vi "CIF_CIPC_Tag Update Test Cases.vi"() -> (0 "error out":errorcluster, 2 "status":string, 3 "pass":bool)   [LabVIEW 2021]
uses:
  <vilib>/CIF Foundation/CIF Channels Core/ChannelCommon/typedef/Direction.ctl
  Double/CIF_CIPC_Chn_Double.lvclass
  C:/Program Files/National Instruments/LabVIEW 2021/vi.lib/CIF Foundation/CIF Channels Core/CIFChannels/CIFChannels.lvclass
  <vilib>/CIF Foundation/CIF Channels Core/ChannelCommon/typedef/New FIFO Instance Response.ctl
  U64/CIF_CIPC_Chn_U64.lvclass
  I64/CIF_CIPC_Chn_I64.lvclass
  a89bac37-e40b-4e23-8b15-caa5b580b70d.vi
  5767d73f-78c6-4091-81b3-8b4b134aad93.vi
  e629907d-3875-4979-a690-95404f934dc5.vi
  a89bac37-e40b-4e23-8b15-caa5b580b70d.vi/49b3dd2d-4579-4089-b72e-3f0875c862f2.vi
  <vilib>/CIF Foundation/CIF CIPC/SubVIs/Check Error.vi
  <vilib>/CIF Foundation/CIF CIPC/SubVIs/Add CIPC Error.vi
  <vilib>/CIF Foundation/CIF CIPC/SubVIs/Get dll Path.vi
  <vilib>/CIF Foundation/CIF CIPC/SubVIs/Notify Of New Write.vi
  <vilib>/CIF Foundation/CIF CIPC/SubVIs/Get Element Write Position.vi
  <vilib>/CIF Foundation/CIF CIPC/SubVIs/Wait For N Elements Available.vi
  <vilib>/CIF Foundation/CIF CIPC/SubVIs/Get Element Read Position.vi
  <vilib>/CIF Foundation/CIF CIPC/SubVIs/Set Element Read Position.vi
  <vilib>/CIF Foundation/CIF CIPC/SubVIs/Get Element Description Variant.vi
  <vilib>/Utility/error.llb/Trim Whitespace.vi
  <vilib>/CIF Foundation/CIF CIPC/SubVIs/Check Error Core.vi
  <vilib>/CIF Foundation/CIF CIPC/SubVIs/Add CIPC Error Core.vi
  <vilib>/CIF Foundation/CIF CIPC/SubVIs/Get Element Info Variant.vi
  <vilib>/CIF Foundation/CIF Channels Core/ChannelCommon/ChannelCommon.lvlib
  <vilib>/CIF Foundation/CIF Channels Core/CIFChannels/CIFChannels.lvclass
  <vilib>/CIF Foundation/CIF CIPC/CIF_NI_CIPC.lvlib
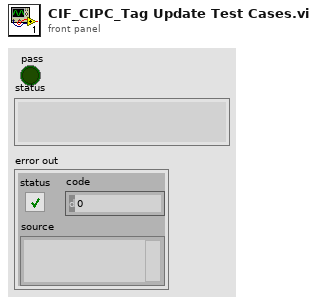
[diagram p1: front panel]
types:
  T1 = typedef "ChannelCommon.lvlib/Direction.ctl" = enum8{"Publisher", "Subscriber"}
  T2 = typedef "ChannelCommon.lvlib/New FIFO Instance Response.ctl" = cluster{"Publisher":string, "Custom Data":u8[]}
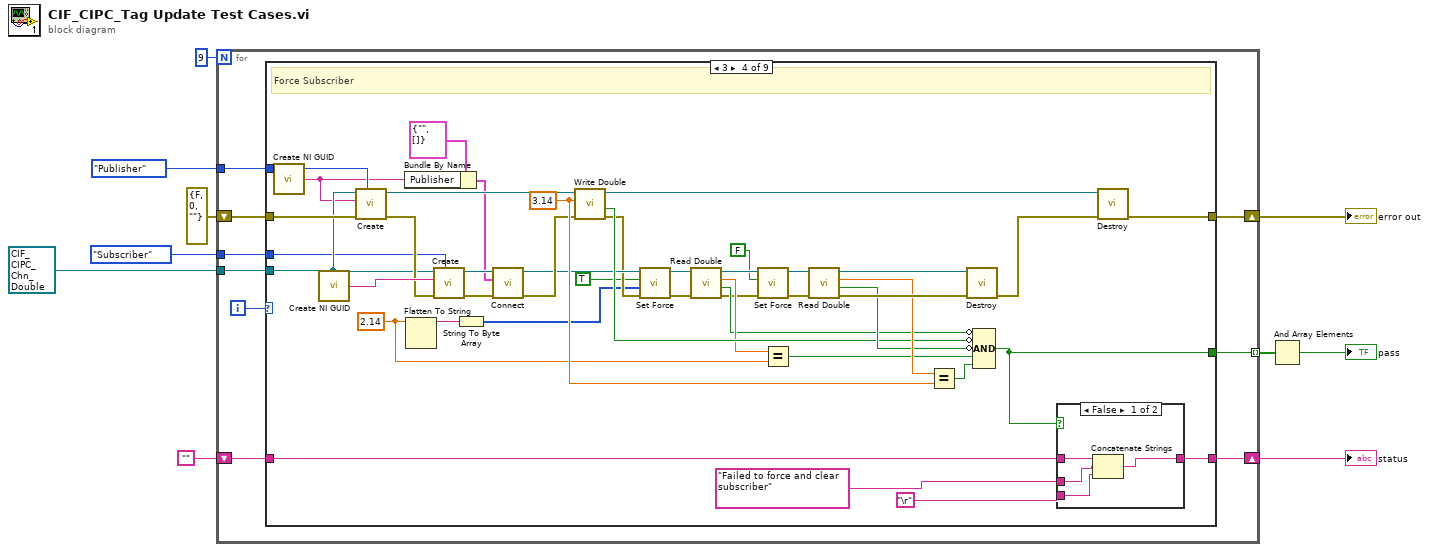
[diagram p0: block diagram]
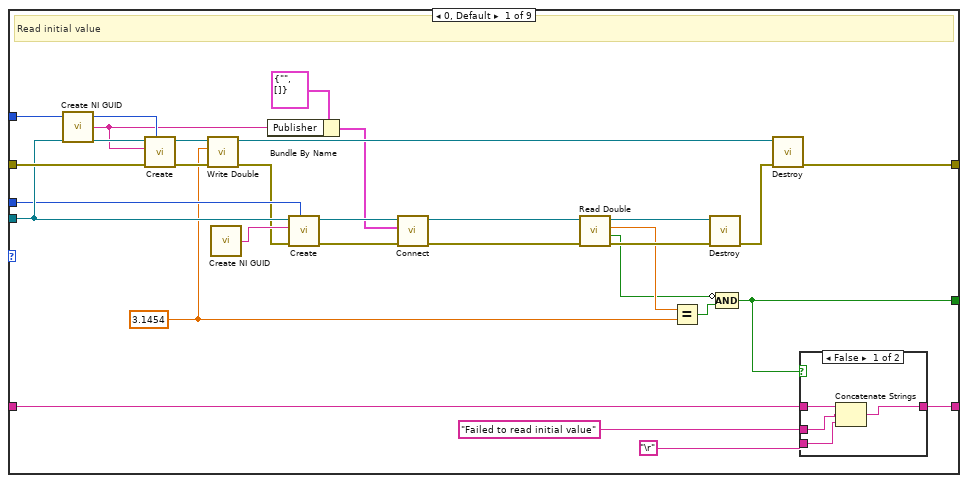
[diagram p2: hidden frame]
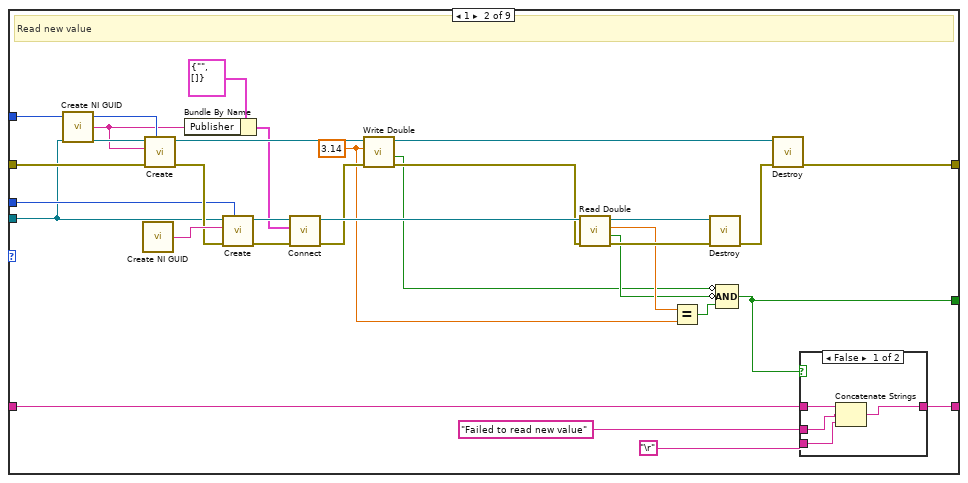
[diagram p4: hidden frame]
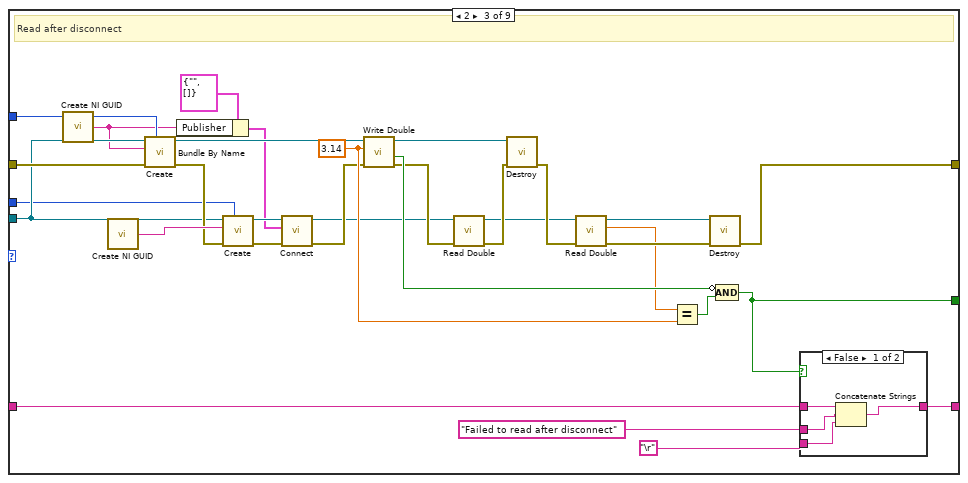
[diagram p6: hidden frame]
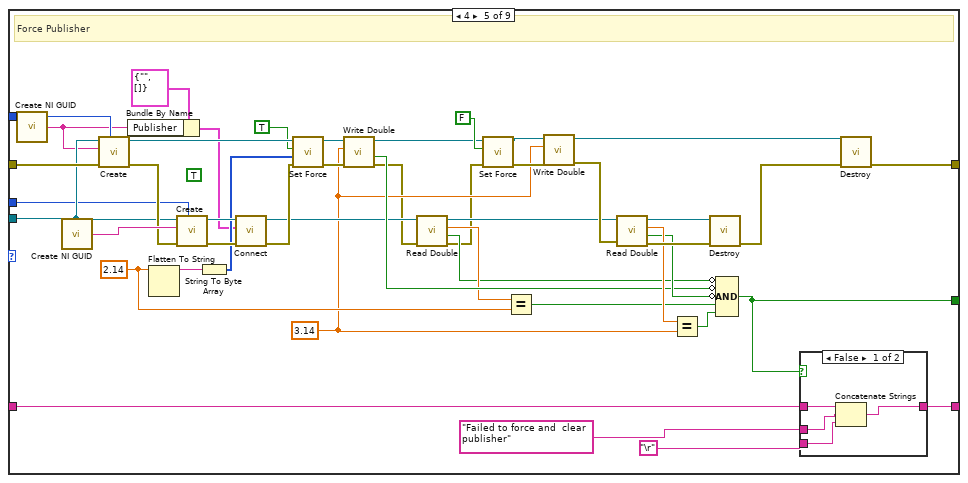
[diagram p9: hidden frame]
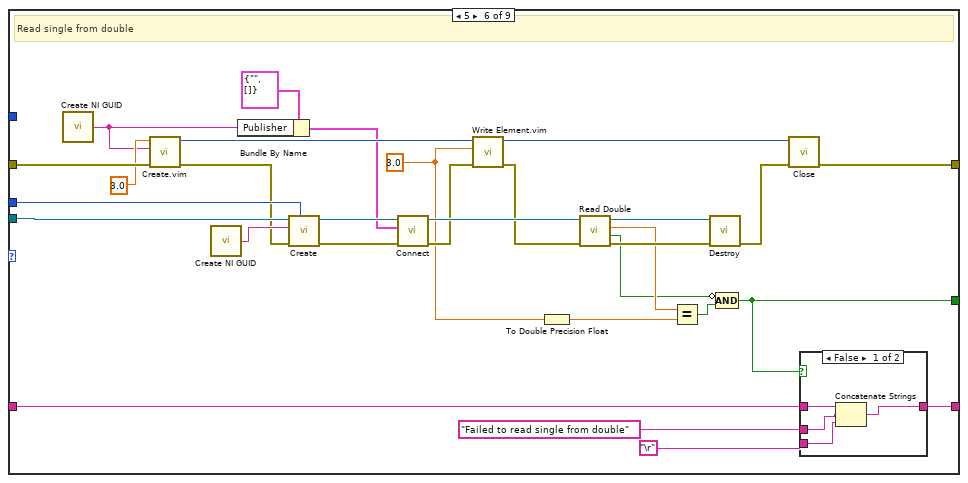
[diagram p11: hidden frame]
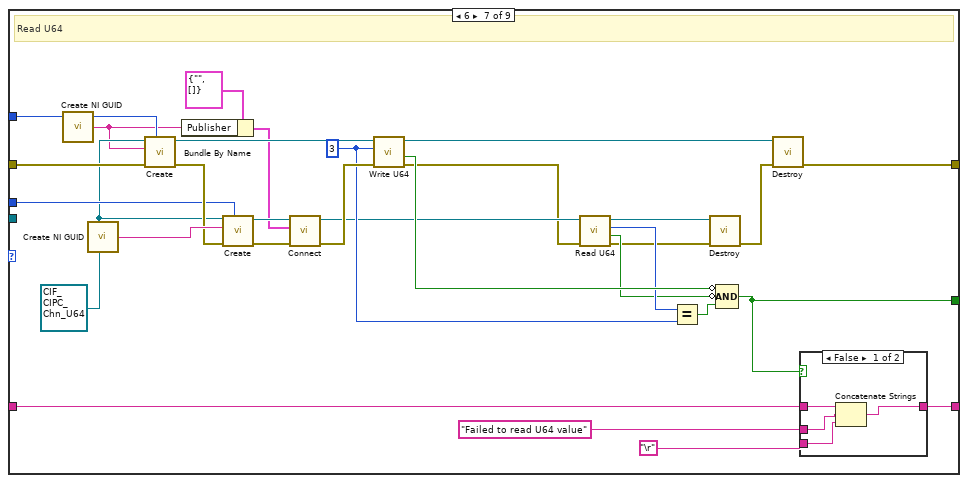
[diagram p13: hidden frame]
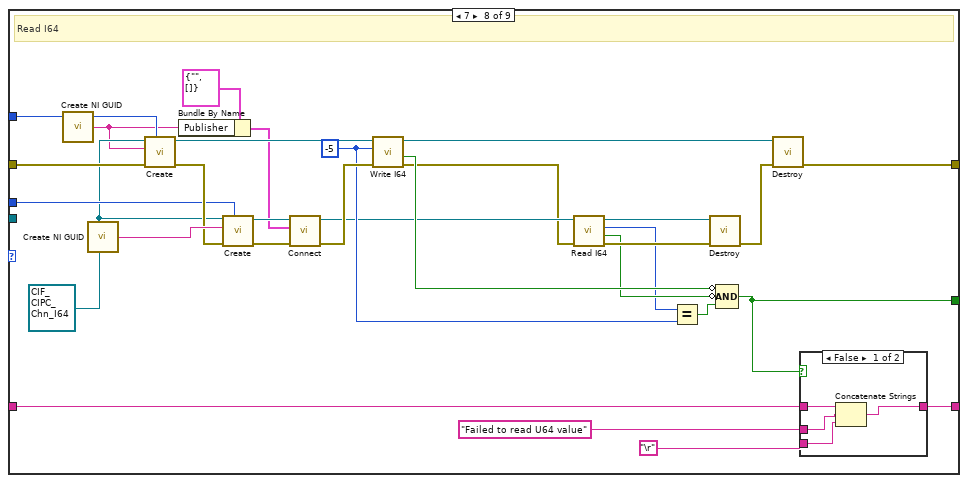
[diagram p15: hidden frame]
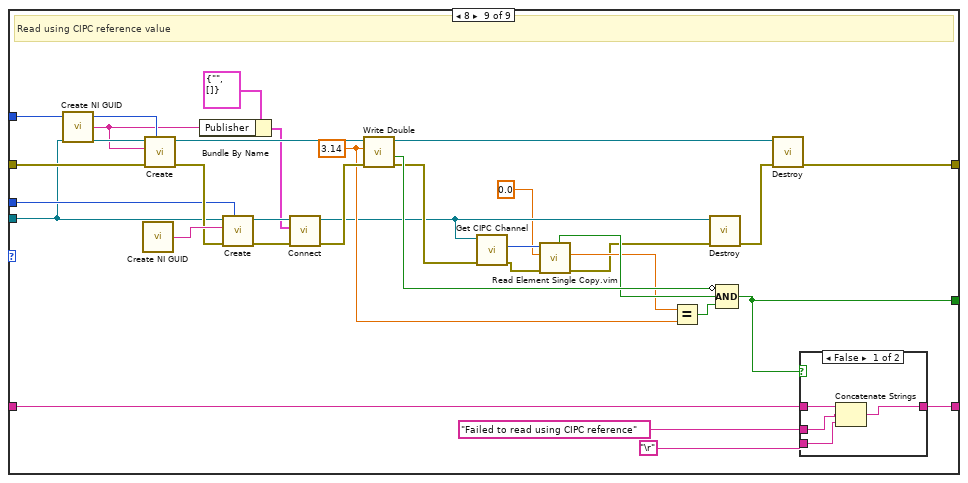
[diagram p17: hidden frame]
diagram:
  n1 = for {
    N: 9 -> [_]
    tunnel: [w19] -> w10 mode=indexing
    shift-right: [w17] -> w5
    shift-left: errorcluster {"status"=FALSE, "code"=0, "source"=""} ("error out") -> [w18]
    shift-right: [w14] -> w6
    shift-left: "" -> [w15]
    tunnel: refnum<class "CIF_CIPC_Chn_Double.lvclass"> refnum ("CIF_CIPC_Chn_Double.lvclass") -> [w13]
    tunnel: Direction."Publisher" ("Direction") -> [w12]
    tunnel: Direction."Subscriber" ("Direction") -> [w11]
    i -> [w16]
    n2 = case shown="3" w16 {
      tunnel: [w32 w67 w111 w158 w209 w242 w277 w312 w349] -> w19
      tunnel: w18 -> [w44 w79 w115 w164 w215 w234 w285 w320 w357]
      tunnel: [w35 w70 w104 w128 w193 w237 w279 w314 w351] -> w17
      tunnel: w15 -> [w48 w83 w119 w168 w219 w254 w289 w324 w361]
      tunnel: [w47 w82 w118 w167 w218 w253 w288 w323 w360] -> w14
      tunnel: w13 -> [w29 w57 w99 w149 w204 w240 _ _ w341]
      tunnel: w12 -> [w30 w59 w98 w148 w203 _ w276 w311 w343]
      tunnel: w11 -> [w28 w58 w97 w147 w202 w239 w275 w310 w342]
      frame 0, Default {
        w23 = 3.1454
        # "Read initial value"
        n3 = call <vilib>:"Create NI GUID.vi"() -> ("NI GUID"=w21:string)
        n4 = call-dynamic "Create.vi"("Direction"=w30, "error in (no error)"=w44, "Name"=w21, "CIFTag in"=w29) -> ("error out"=w26:errorcluster, "CIFTag out"=w27:refnum<class "CIF_CIPC_Chn_Double.lvclass">)  [unwired: 6 in]
        n5 = call-dynamic "Write Double.vi"("error in (no error)"=w26, "Data"=w23, "CIFTag in"=w27) -> ("error out"=w24:errorcluster, "CIFTag out"=w25:refnum<class "CIF_CIPC_Chn_Double.lvclass">)  [unwired: 6 in, 1 out]
        n6 = call <vilib>:"Create NI GUID.vi"() -> ("NI GUID"=w43:string)
        n7 = Bundle By Name(cluster=T2 {"Publisher"="", "Custom Data"=[]} ("Connection"), "Publisher"=w21) -> (w20:T2)
        n8 = call-dynamic "Create.vi"("Direction"=w28, "error in (no error)"=w24, "Name"=w43, "CIFTag in"=w29) -> ("error out"=w41:errorcluster, "CIFTag out"=w42:refnum<class "CIF_CIPC_Chn_Double.lvclass">)  [unwired: 6 in]
        n9 = call-dynamic "Connect.vi"("error in (no error)"=w41, "Connection"=w20, "CIFTag in"=w42) -> ("error out"=w39:errorcluster, "CIFTag out"=w40:refnum<class "CIF_CIPC_Chn_Double.lvclass">)  [unwired: 7 in]
        n10 = call-dynamic "Read Double.vi"("error in (no error)"=w39, "CIFTag in"=w40) -> ("error out"=w37:errorcluster, "timed out?"=w31:bool, "Data"=w34:dbl, "CIFTag out"=w38:refnum<class "CIF_CIPC_Chn_Double.lvclass">)  [unwired: 6 in]
        n11 = Equal?(x=w34, y=w23) -> (x = y?=w33:bool)
        n12 = call-dynamic "Destroy.vi"("error in (no error)"=w37, "CIFTag in"=w38) -> ("error out"=w36:errorcluster)  [unwired: 8 in, 1 out]
        n13 = Compound Arithmetic op=AND(invert w31, w33) -> (w32:bool)
        n14 = call-dynamic "Destroy.vi"("error in (no error)"=w36, "CIFTag in"=w25) -> ("error out"=w35:errorcluster)  [unwired: 8 in, 1 out]
        n15 = case shown="False" w32 {
          tunnel: w48 -> [w52 w53]
          tunnel: [w49 w53] -> w47
          tunnel: "Failed to read initial value" -> [w51 _]
          tunnel: "\r" -> [w50 _]
          frame False {
            n16 = Concatenate Strings(w52, w51, w50) -> (w49:string)
          }
          frame True {
          }
        }
      }
      frame 1 {
        w60 = 3.14 ("Data")
        # "Read new value"
        n17 = call <vilib>:"Create NI GUID.vi"() -> ("NI GUID"=w55:string)
        n18 = call <vilib>:"Create NI GUID.vi"() -> ("NI GUID"=w78:string)
        n19 = call-dynamic "Create.vi"("Direction"=w59, "error in (no error)"=w79, "Name"=w55, "CIFTag in"=w57) -> ("error out"=w77:errorcluster, "CIFTag out"=w65:refnum<class "CIF_CIPC_Chn_Double.lvclass">)  [unwired: 6 in]
        n20 = Bundle By Name(cluster=T2 {"Publisher"="", "Custom Data"=[]} ("Connection"), "Publisher"=w55) -> (w54:T2)
        n21 = call-dynamic "Create.vi"("Direction"=w58, "error in (no error)"=w77, "Name"=w78, "CIFTag in"=w57) -> ("error out"=w75:errorcluster, "CIFTag out"=w76:refnum<class "CIF_CIPC_Chn_Double.lvclass">)  [unwired: 6 in]
        n22 = call-dynamic "Connect.vi"("error in (no error)"=w75, "Connection"=w54, "CIFTag in"=w76) -> ("error out"=w64:errorcluster, "CIFTag out"=w74:refnum<class "CIF_CIPC_Chn_Double.lvclass">)  [unwired: 7 in]
        n23 = call-dynamic "Write Double.vi"("error in (no error)"=w64, "Data"=w60, "CIFTag in"=w65) -> ("error out"=w63:errorcluster, "timed out?"=w61:bool, "CIFTag out"=w62:refnum<class "CIF_CIPC_Chn_Double.lvclass">)  [unwired: 6 in]
        n24 = call-dynamic "Read Double.vi"("error in (no error)"=w63, "CIFTag in"=w74) -> ("error out"=w72:errorcluster, "timed out?"=w66:bool, "Data"=w69:dbl, "CIFTag out"=w73:refnum<class "CIF_CIPC_Chn_Double.lvclass">)  [unwired: 6 in]
        n25 = Equal?(x=w69, y=w60) -> (x = y?=w68:bool)
        n26 = call-dynamic "Destroy.vi"("error in (no error)"=w72, "CIFTag in"=w73) -> ("error out"=w71:errorcluster)  [unwired: 8 in, 1 out]
        n27 = Compound Arithmetic op=AND(invert w61, invert w66, w68) -> (w67:bool)
        n28 = call-dynamic "Destroy.vi"("error in (no error)"=w71, "CIFTag in"=w62) -> ("error out"=w70:errorcluster)  [unwired: 8 in, 1 out]
        n29 = case shown="False" w67 {
          tunnel: w83 -> [w87 w88]
          tunnel: [w84 w88] -> w82
          tunnel: "Failed to read new value" -> [w86 _]
          tunnel: "\r" -> [w85 _]
          frame False {
            n30 = Concatenate Strings(w87, w86, w85) -> (w84:string)
          }
          frame True {
          }
        }
      }
      frame 2 {
        w105 = 3.14 ("Data")
        # "Read after disconnect"
        n31 = call <vilib>:"Create NI GUID.vi"() -> ("NI GUID"=w90:string)
        n32 = call <vilib>:"Create NI GUID.vi"() -> ("NI GUID"=w114:string)
        n33 = call-dynamic "Create.vi"("Direction"=w98, "error in (no error)"=w115, "Name"=w90, "CIFTag in"=w99) -> ("error out"=w113:errorcluster, "CIFTag out"=w110:refnum<class "CIF_CIPC_Chn_Double.lvclass">)  [unwired: 6 in]
        n34 = Bundle By Name(cluster=T2 {"Publisher"="", "Custom Data"=[]} ("Connection"), "Publisher"=w90) -> (w89:T2)
        n35 = call-dynamic "Create.vi"("Direction"=w97, "error in (no error)"=w113, "Name"=w114, "CIFTag in"=w99) -> ("error out"=w102:errorcluster, "CIFTag out"=w103:refnum<class "CIF_CIPC_Chn_Double.lvclass">)  [unwired: 6 in]
        n36 = call-dynamic "Connect.vi"("error in (no error)"=w102, "Connection"=w89, "CIFTag in"=w103) -> ("error out"=w101:errorcluster, "CIFTag out"=w100:refnum<class "CIF_CIPC_Chn_Double.lvclass">)  [unwired: 7 in]
        n37 = call-dynamic "Write Double.vi"("error in (no error)"=w101, "Data"=w105, "CIFTag in"=w110) -> ("error out"=w108:errorcluster, "timed out?"=w109:bool, "CIFTag out"=w107:refnum<class "CIF_CIPC_Chn_Double.lvclass">)  [unwired: 6 in]
        n38 = call-dynamic "Read Double.vi"("error in (no error)"=w108, "CIFTag in"=w100) -> ("error out"=w106:errorcluster, "CIFTag out"=w95:refnum<class "CIF_CIPC_Chn_Double.lvclass">)  [unwired: 6 in, 2 out]
        n39 = call-dynamic "Destroy.vi"("error in (no error)"=w106, "CIFTag in"=w107) -> ("error out"=w96:errorcluster)  [unwired: 8 in, 1 out]
        n40 = call-dynamic "Read Double.vi"("error in (no error)"=w96, "CIFTag in"=w95) -> ("error out"=w94:errorcluster, "Data"=w93:dbl, "CIFTag out"=w92:refnum<class "CIF_CIPC_Chn_Double.lvclass">)  [unwired: 6 in, 1 out]
        n41 = Equal?(x=w93, y=w105) -> (x = y?=w112:bool)
        n42 = call-dynamic "Destroy.vi"("error in (no error)"=w94, "CIFTag in"=w92) -> ("error out"=w104:errorcluster)  [unwired: 8 in, 1 out]
        n43 = Compound Arithmetic op=AND(invert w109, w112) -> (w111:bool)
        n44 = case shown="False" w111 {
          tunnel: w119 -> [w123 w124]
          tunnel: [w120 w124] -> w118
          tunnel: "Failed to read after disconnect" -> [w122 _]
          tunnel: "\r" -> [w121 _]
          frame False {
            n45 = Concatenate Strings(w123, w122, w121) -> (w120:string)
          }
          frame True {
          }
        }
      }
      frame 3 {
        w138 = 2.14 ("Data")
        w153 = 3.14 ("Data")
        # "Force Subscriber"
        n46 = call <vilib>:"Create NI GUID.vi"() -> ("NI GUID"=w126:string)
        n47 = call <vilib>:"Create NI GUID.vi"() -> ("NI GUID"=w163:string)
        n48 = call-dynamic "Create.vi"("Direction"=w148, "error in (no error)"=w164, "Name"=w126, "CIFTag in"=w149) -> ("error out"=w162:errorcluster, "CIFTag out"=w156:refnum<class "CIF_CIPC_Chn_Double.lvclass">)  [unwired: 6 in]
        n49 = Bundle By Name(cluster=T2 {"Publisher"="", "Custom Data"=[]} ("Connection"), "Publisher"=w126) -> (w125:T2)
        n50 = Flatten To String(anything=w138) -> (data string=w144:string)  [unwired: 3 in, 2 out]
        n51 = call-dynamic "Create.vi"("Direction"=w147, "error in (no error)"=w162, "Name"=w163, "CIFTag in"=w149) -> ("error out"=w151:errorcluster, "CIFTag out"=w152:refnum<class "CIF_CIPC_Chn_Double.lvclass">)  [unwired: 6 in]
        n52 = String To Byte Array(string=w144) -> (unsigned byte array=w143:u8[])
        n53 = call-dynamic "Connect.vi"("error in (no error)"=w151, "Connection"=w125, "CIFTag in"=w152) -> ("error out"=w150:errorcluster, "CIFTag out"=w146:refnum<class "CIF_CIPC_Chn_Double.lvclass">)  [unwired: 7 in]
        n54 = call-dynamic "Write Double.vi"("error in (no error)"=w150, "Data"=w153, "CIFTag in"=w156) -> ("error out"=w145:errorcluster, "timed out?"=w155:bool, "CIFTag out"=w154:refnum<class "CIF_CIPC_Chn_Double.lvclass">)  [unwired: 6 in]
        n55 = call <vilib>:"Set Force.vi"("error in (no error)"=w145, "Force Data"=w143, "Force Active"=TRUE, "CIFChannels in"=w146) -> ("error out"=w140:errorcluster, "CIFChannels out"=w141:refnum<class "CIF_CIPC_Chn_Double.lvclass">)  [unwired: 6 in]
        n56 = call-dynamic "Read Double.vi"("error in (no error)"=w140, "CIFTag in"=w141) -> ("error out"=w133:errorcluster, "timed out?"=w137:bool, "Data"=w139:dbl, "CIFTag out"=w134:refnum<class "CIF_CIPC_Chn_Double.lvclass">)  [unwired: 6 in]
        n57 = call <vilib>:"Set Force.vi"("error in (no error)"=w133, "Force Active"=FALSE, "CIFChannels in"=w134) -> ("error out"=w132:errorcluster, "CIFChannels out"=w131:refnum<class "CIF_CIPC_Chn_Double.lvclass">)  [unwired: 7 in]
        n58 = Equal?(x=w139, y=w138) -> (x = y?=w135:bool)
        n59 = call-dynamic "Read Double.vi"("error in (no error)"=w132, "CIFTag in"=w131) -> ("error out"=w160:errorcluster, "timed out?"=w157:bool, "Data"=w159:dbl, "CIFTag out"=w161:refnum<class "CIF_CIPC_Chn_Double.lvclass">)  [unwired: 6 in]
        n60 = Equal?(x=w159, y=w153) -> (x = y?=w136:bool)
        n61 = call-dynamic "Destroy.vi"("error in (no error)"=w160, "CIFTag in"=w161) -> ("error out"=w129:errorcluster)  [unwired: 8 in, 1 out]
        n62 = Compound Arithmetic op=AND(invert w137, invert w155, invert w157, w135, w136) -> (w158:bool)
        n63 = case shown="False" w158 {
          tunnel: w168 -> [w172 w173]
          tunnel: [w169 w173] -> w167
          tunnel: "Failed to force and clear subscriber" -> [w171 _]
          tunnel: "\r" -> [w170 _]
          frame False {
            n64 = Concatenate Strings(w172, w171, w170) -> (w169:string)
          }
          frame True {
          }
        }
        n65 = call-dynamic "Destroy.vi"("error in (no error)"=w129, "CIFTag in"=w154) -> ("error out"=w128:errorcluster)  [unwired: 8 in, 1 out]
      }
      frame 4 {
        (unwired) TRUE ("Force Active")
        w199 = 2.14 ("Data")
        w182 = 3.14 ("Data")
        # "Force Publisher"
        n66 = call <vilib>:"Create NI GUID.vi"() -> ("NI GUID"=w175:string)
        n67 = call <vilib>:"Create NI GUID.vi"() -> ("NI GUID"=w214:string)
        n68 = call-dynamic "Create.vi"("Direction"=w203, "error in (no error)"=w215, "Name"=w175, "CIFTag in"=w204) -> ("error out"=w213:errorcluster, "CIFTag out"=w192:refnum<class "CIF_CIPC_Chn_Double.lvclass">)  [unwired: 6 in]
        n69 = Bundle By Name(cluster=T2 {"Publisher"="", "Custom Data"=[]} ("Connection"), "Publisher"=w175) -> (w174:T2)
        n70 = Flatten To String(anything=w199) -> (data string=w201:string)  [unwired: 3 in, 2 out]
        n71 = call-dynamic "Create.vi"("Direction"=w202, "error in (no error)"=w213, "Name"=w214, "CIFTag in"=w204) -> ("error out"=w205:errorcluster, "CIFTag out"=w206:refnum<class "CIF_CIPC_Chn_Double.lvclass">)  [unwired: 6 in]
        n72 = String To Byte Array(string=w201) -> (unsigned byte array=w191:u8[])
        n73 = call-dynamic "Connect.vi"("error in (no error)"=w205, "Connection"=w174, "CIFTag in"=w206) -> ("error out"=w188:errorcluster, "CIFTag out"=w186:refnum<class "CIF_CIPC_Chn_Double.lvclass">)  [unwired: 7 in]
        n74 = call <vilib>:"Set Force.vi"("error in (no error)"=w188, "Force Data"=w191, "Force Active"=TRUE, "CIFChannels in"=w192) -> ("error out"=w189:errorcluster, "CIFChannels out"=w190:refnum<class "CIF_CIPC_Chn_Double.lvclass">)  [unwired: 6 in]
        n75 = call-dynamic "Write Double.vi"("error in (no error)"=w189, "Data"=w182, "CIFTag in"=w190) -> ("error out"=w178:errorcluster, "timed out?"=w207:bool, "CIFTag out"=w185:refnum<class "CIF_CIPC_Chn_Double.lvclass">)  [unwired: 6 in]
        n76 = call-dynamic "Read Double.vi"("error in (no error)"=w178, "CIFTag in"=w186) -> ("error out"=w177:errorcluster, "timed out?"=w198:bool, "Data"=w200:dbl, "CIFTag out"=w179:refnum<class "CIF_CIPC_Chn_Double.lvclass">)  [unwired: 6 in]
        n77 = call <vilib>:"Set Force.vi"("error in (no error)"=w177, "Force Active"=FALSE, "CIFChannels in"=w185) -> ("error out"=w184:errorcluster, "CIFChannels out"=w183:refnum<class "CIF_CIPC_Chn_Double.lvclass">)  [unwired: 7 in]
        n78 = Equal?(x=w200, y=w199) -> (x = y?=w196:bool)
        n79 = call-dynamic "Write Double.vi"("error in (no error)"=w184, "Data"=w182, "CIFTag in"=w183) -> ("error out"=w181:errorcluster, "CIFTag out"=w180:refnum<class "CIF_CIPC_Chn_Double.lvclass">)  [unwired: 6 in, 1 out]
        n80 = call-dynamic "Read Double.vi"("error in (no error)"=w181, "CIFTag in"=w179) -> ("error out"=w211:errorcluster, "timed out?"=w208:bool, "Data"=w210:dbl, "CIFTag out"=w212:refnum<class "CIF_CIPC_Chn_Double.lvclass">)  [unwired: 6 in]
        n81 = Equal?(x=w210, y=w182) -> (x = y?=w197:bool)
        n82 = call-dynamic "Destroy.vi"("error in (no error)"=w211, "CIFTag in"=w212) -> ("error out"=w194:errorcluster)  [unwired: 8 in, 1 out]
        n83 = Compound Arithmetic op=AND(invert w198, invert w207, invert w208, w196, w197) -> (w209:bool)
        n84 = case shown="False" w209 {
          tunnel: w219 -> [w223 w224]
          tunnel: [w220 w224] -> w218
          tunnel: "Failed to force and  clear publisher" -> [w222 _]
          tunnel: "\r" -> [w221 _]
          frame False {
            n85 = Concatenate Strings(w223, w222, w221) -> (w220:string)
          }
          frame True {
          }
        }
        n86 = call-dynamic "Destroy.vi"("error in (no error)"=w194, "CIFTag in"=w180) -> ("error out"=w193:errorcluster)  [unwired: 8 in, 1 out]
      }
      frame 5 {
        w230 = sgl 3.0
        # "Read single from double"
        n87 = call <vilib>:"Create NI GUID.vi"() -> ("NI GUID"=w226:string)
        n88 = call "Create.vim"("error in (no error)"=w234, "Name in"=w226, "Data Type"=sgl 3.0) -> ("error out"=w232:errorcluster, "CIPC Reference"=w231:u64)  [unwired: 5 in, 2 out]
        n89 = call <vilib>:"Create NI GUID.vi"() -> ("NI GUID"=w250:string)
        n90 = Bundle By Name(cluster=T2 {"Publisher"="", "Custom Data"=[]} ("Connection"), "Publisher"=w226) -> (w225:T2)
        n91 = call-dynamic "Create.vi"("Direction"=w239, "error in (no error)"=w232, "Name"=w250, "CIFTag in"=w240) -> ("error out"=w248:errorcluster, "CIFTag out"=w249:refnum<class "CIF_CIPC_Chn_Double.lvclass">)  [unwired: 6 in]
        n92 = call-dynamic "Connect.vi"("error in (no error)"=w248, "Connection"=w225, "CIFTag in"=w249) -> ("error out"=w236:errorcluster, "CIFTag out"=w247:refnum<class "CIF_CIPC_Chn_Double.lvclass">)  [unwired: 7 in]
        n93 = call "Write Element.vim"("error in (no error)"=w236, "Data in"=w230, "CIPC Reference in"=w231) -> ("error out"=w235:errorcluster, "CIPC Reference out"=w229:u64)  [unwired: 5 in, 2 out]
        n94 = To Double Precision Float(number=w230) -> (double precision float=w228:dbl)
        n95 = call-dynamic "Read Double.vi"("error in (no error)"=w235, "CIFTag in"=w247) -> ("error out"=w245:errorcluster, "timed out?"=w241:bool, "Data"=w244:dbl, "CIFTag out"=w246:refnum<class "CIF_CIPC_Chn_Double.lvclass">)  [unwired: 6 in]
        n96 = Equal?(x=w244, y=w228) -> (x = y?=w243:bool)
        n97 = call-dynamic "Destroy.vi"("error in (no error)"=w245, "CIFTag in"=w246) -> ("error out"=w238:errorcluster)  [unwired: 8 in, 1 out]
        n98 = Compound Arithmetic op=AND(invert w241, w243) -> (w242:bool)
        n99 = call <vilib>:"Close.vi"("error in (no error)"=w238, "CIPC Reference"=w229) -> ("error out"=w237:errorcluster)  [unwired: 9 in]
        n100 = case shown="False" w242 {
          tunnel: w254 -> [w258 w259]
          tunnel: [w255 w259] -> w253
          tunnel: "Failed to read single from double" -> [w257 _]
          tunnel: "\r" -> [w256 _]
          frame False {
            n101 = Concatenate Strings(w258, w257, w256) -> (w255:string)
          }
          frame True {
          }
        }
      }
      frame 6 {
        w274 = refnum<class "CIF_CIPC_Chn_U64.lvclass"> refnum ("CIF_CIPC_Chn_U64.lvclass")
        w269 = u64 3 ("Data")
        # "Read U64"
        n102 = call <vilib>:"Create NI GUID.vi"() -> ("NI GUID"=w261:string)
        n103 = call <vilib>:"Create NI GUID.vi"() -> ("NI GUID"=w284:string)
        n104 = call-dynamic "Create.vi"("Direction"=w276, "error in (no error)"=w285, "Name"=w261, "CIFTag in"=w274) -> ("error out"=w283:errorcluster, "CIFTag out"=w272:refnum<class "CIF_CIPC_Chn_U64.lvclass">)  [unwired: 6 in]
        n105 = Bundle By Name(cluster=T2 {"Publisher"="", "Custom Data"=[]} ("Connection"), "Publisher"=w261) -> (w260:T2)
        n106 = call-dynamic "Create.vi"("Direction"=w275, "error in (no error)"=w283, "Name"=w284, "CIFTag in"=w274) -> ("error out"=w281:errorcluster, "CIFTag out"=w282:refnum<class "CIF_CIPC_Chn_U64.lvclass">)  [unwired: 6 in]
        n107 = call-dynamic "Connect.vi"("error in (no error)"=w281, "Connection"=w260, "CIFTag in"=w282) -> ("error out"=w273:errorcluster, "CIFTag out"=w268:refnum<class "CIF_CIPC_Chn_U64.lvclass">)  [unwired: 7 in]
        n108 = call-dynamic "Write U64.vi"("error in (no error)"=w273, "Data"=w269, "CIFTag in"=w272) -> ("error out"=w267:errorcluster, "timed out?"=w270:bool, "CIFTag out"=w271:refnum<class "CIF_CIPC_Chn_U64.lvclass">)  [unwired: 6 in]
        n109 = call-dynamic "Read U64.vi"("error in (no error)"=w267, "CIFTag in"=w268) -> ("error out"=w263:errorcluster, "timed out?"=w264:bool, "Data"=w265:u64, "CIFTag out"=w266:refnum<class "CIF_CIPC_Chn_U64.lvclass">)  [unwired: 6 in]
        n110 = Equal?(x=w265, y=w269) -> (x = y?=w278:bool)
        n111 = call-dynamic "Destroy.vi"("error in (no error)"=w263, "CIFTag in"=w266) -> ("error out"=w280:errorcluster)  [unwired: 8 in, 1 out]
        n112 = Compound Arithmetic op=AND(invert w270, invert w264, w278) -> (w277:bool)
        n113 = call-dynamic "Destroy.vi"("error in (no error)"=w280, "CIFTag in"=w271) -> ("error out"=w279:errorcluster)  [unwired: 8 in, 1 out]
        n114 = case shown="False" w277 {
          tunnel: w289 -> [w293 w294]
          tunnel: [w290 w294] -> w288
          tunnel: "Failed to read U64 value" -> [w292 _]
          tunnel: "\r" -> [w291 _]
          frame False {
            n115 = Concatenate Strings(w293, w292, w291) -> (w290:string)
          }
          frame True {
          }
        }
      }
      frame 7 {
        w298 = refnum<class "CIF_CIPC_Chn_I64.lvclass"> refnum ("CIF_CIPC_Chn_I64.lvclass")
        w307 = i64 -5 ("Data")
        # "Read I64"
        n116 = call <vilib>:"Create NI GUID.vi"() -> ("NI GUID"=w296:string)
        n117 = call <vilib>:"Create NI GUID.vi"() -> ("NI GUID"=w319:string)
        n118 = call-dynamic "Create.vi"("Direction"=w311, "error in (no error)"=w320, "Name"=w296, "CIFTag in"=w298) -> ("error out"=w318:errorcluster, "CIFTag out"=w309:refnum<class "CIF_CIPC_Chn_I64.lvclass">)  [unwired: 6 in]
        n119 = Bundle By Name(cluster=T2 {"Publisher"="", "Custom Data"=[]} ("Connection"), "Publisher"=w296) -> (w295:T2)
        n120 = call-dynamic "Create.vi"("Direction"=w310, "error in (no error)"=w318, "Name"=w319, "CIFTag in"=w298) -> ("error out"=w316:errorcluster, "CIFTag out"=w317:refnum<class "CIF_CIPC_Chn_I64.lvclass">)  [unwired: 6 in]
        n121 = call-dynamic "Connect.vi"("error in (no error)"=w316, "Connection"=w295, "CIFTag in"=w317) -> ("error out"=w308:errorcluster, "CIFTag out"=w304:refnum<class "CIF_CIPC_Chn_I64.lvclass">)  [unwired: 7 in]
        n122 = call-dynamic "Write I64.vi"("error in (no error)"=w308, "Data"=w307, "CIFTag in"=w309) -> ("error out"=w303:errorcluster, "timed out?"=w305:bool, "CIFTag out"=w306:refnum<class "CIF_CIPC_Chn_I64.lvclass">)  [unwired: 6 in]
        n123 = call-dynamic "Read I64.vi"("error in (no error)"=w303, "CIFTag in"=w304) -> ("error out"=w302:errorcluster, "timed out?"=w301:bool, "Data"=w300:i64, "CIFTag out"=w299:refnum<class "CIF_CIPC_Chn_I64.lvclass">)  [unwired: 6 in]
        n124 = Equal?(x=w300, y=w307) -> (x = y?=w313:bool)
        n125 = call-dynamic "Destroy.vi"("error in (no error)"=w302, "CIFTag in"=w299) -> ("error out"=w315:errorcluster)  [unwired: 8 in, 1 out]
        n126 = Compound Arithmetic op=AND(invert w305, invert w301, w313) -> (w312:bool)
        n127 = call-dynamic "Destroy.vi"("error in (no error)"=w315, "CIFTag in"=w306) -> ("error out"=w314:errorcluster)  [unwired: 8 in, 1 out]
        n128 = case shown="False" w312 {
          tunnel: w324 -> [w328 w329]
          tunnel: [w325 w329] -> w323
          tunnel: "Failed to read U64 value" -> [w327 _]
          tunnel: "\r" -> [w326 _]
          frame False {
            n129 = Concatenate Strings(w328, w327, w326) -> (w325:string)
          }
          frame True {
          }
        }
      }
      frame 8 {
        w344 = 3.14 ("Data")
        # "Read using CIPC reference value"
        n130 = call <vilib>:"Create NI GUID.vi"() -> ("NI GUID"=w331:string)
        n131 = call <vilib>:"Create NI GUID.vi"() -> ("NI GUID"=w356:string)
        n132 = call-dynamic "Create.vi"("Direction"=w343, "error in (no error)"=w357, "Name"=w331, "CIFTag in"=w341) -> ("error out"=w355:errorcluster, "CIFTag out"=w348:refnum<class "CIF_CIPC_Chn_Double.lvclass">)  [unwired: 6 in]
        n133 = Bundle By Name(cluster=T2 {"Publisher"="", "Custom Data"=[]} ("Connection"), "Publisher"=w331) -> (w330:T2)
        n134 = call-dynamic "Create.vi"("Direction"=w342, "error in (no error)"=w355, "Name"=w356, "CIFTag in"=w341) -> ("error out"=w353:errorcluster, "CIFTag out"=w354:refnum<class "CIF_CIPC_Chn_Double.lvclass">)  [unwired: 6 in]
        n135 = call-dynamic "Connect.vi"("error in (no error)"=w353, "Connection"=w330, "CIFTag in"=w354) -> ("error out"=w347:errorcluster, "CIFTag out"=w339:refnum<class "CIF_CIPC_Chn_Double.lvclass">)  [unwired: 7 in]
        n136 = call-dynamic "Write Double.vi"("error in (no error)"=w347, "Data"=w344, "CIFTag in"=w348) -> ("error out"=w340:errorcluster, "timed out?"=w345:bool, "CIFTag out"=w346:refnum<class "CIF_CIPC_Chn_Double.lvclass">)  [unwired: 6 in]
        n137 = call-dynamic "Get CIPC Channel.vi"("error in (no error)"=w340, "CIF_CIPC_Chn in"=w339) -> ("error out"=w333:errorcluster, "CIPC Channel"=w338:u64)  [unwired: 7 in, 1 out]
        n138 = call "Read Element Single Copy.vim"("error in (no error)"=w333, "Data in"=0.0 ("Data"), "CIPC Reference in"=w338) -> ("error out"=w334:errorcluster, "Data out"=w335:dbl, "Success"=w336:bool)  [unwired: 4 in, 2 out]
        n139 = Equal?(x=w335, y=w344) -> (x = y?=w350:bool)
        n140 = call-dynamic "Destroy.vi"("error in (no error)"=w334, "CIFTag in"=w339) -> ("error out"=w352:errorcluster)  [unwired: 8 in, 1 out]
        n141 = Compound Arithmetic op=AND(invert w345, w336, w350) -> (w349:bool)
        n142 = call-dynamic "Destroy.vi"("error in (no error)"=w352, "CIFTag in"=w346) -> ("error out"=w351:errorcluster)  [unwired: 8 in, 1 out]
        n143 = case shown="False" w349 {
          tunnel: w361 -> [w365 w366]
          tunnel: [w362 w366] -> w360
          tunnel: "Failed to read using CIPC reference" -> [w364 _]
          tunnel: "\r" -> [w363 _]
          frame False {
            n144 = Concatenate Strings(w365, w364, w363) -> (w362:string)
          }
          frame True {
          }
        }
      }
    }
  }
  "error out" <- w5
  "status" <- w6
  n145 = And Array Elements(Boolean array=w10) -> (logical AND=→"pass":bool)
